vi "ReadName.vi"(8 "error in (no error)":errorcluster, 11 "object in":refnum<class "Configuration.lvclass">) -> (0 "error out":errorcluster, 2 "Name":string, 3 "object out":refnum<class "Configuration.lvclass">)   [LabVIEW 2021, in "Channel.lvlib" / "Configuration.lvclass"]
uses:
  Configuration.lvclass
  Configuration.lvclass/Configuration.ctl
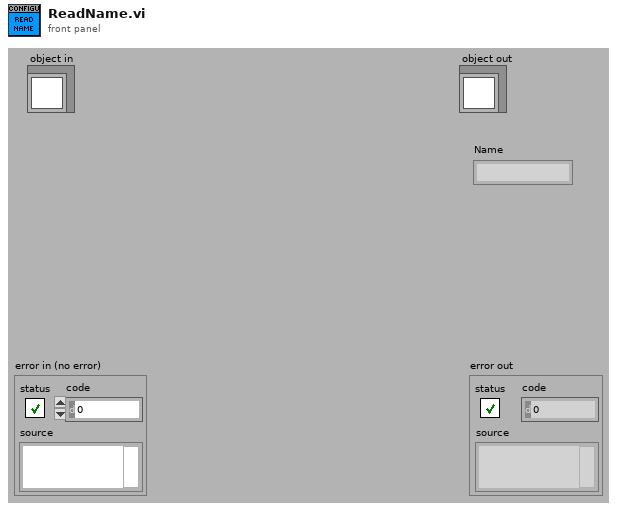
[diagram p1: front panel]
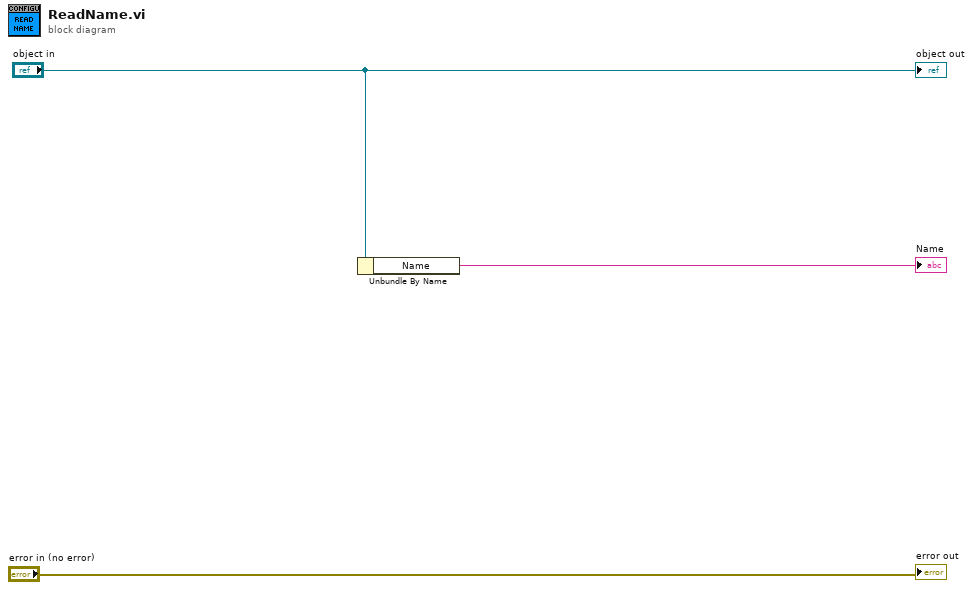
[diagram p0: block diagram]
diagram:
  n1 = Unbundle By Name("object in") -> ("Name"=→"Name":string)
  "error out" <- "error in (no error)"
  "object out" <- "object in"
